vi "Create Wrapper for Code Module - Multiple Convertervi.vi"(11 "error in":errorcluster) -> (15 "error out":errorcluster)   [LabVIEW 2021, in "Converter.lvlib"]
uses:
  Converter.lvlib
  <vilib>/Utility/miscctls.llb/LVPointTypeDef.ctl
  <vilib>/Utility/traverseref.llb/TRef TravTarget.ctl
  <vilib>/Utility/traverseref.llb/VI Scripting - Traverse.lvlib
  Converter Reusables/Converter Reusables.lvlib
  Path Functions/Path Functions.lvlib
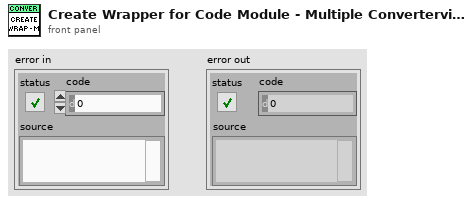
[diagram p1: front panel]
types:
  T1 = typedef "TRef TravTarget.ctl" = enum16{"FP", "BD", "Other"}
  T2 = typedef "LVPointTypeDef.ctl" = cluster{"Horizontal":i16, "Vertical":i16}
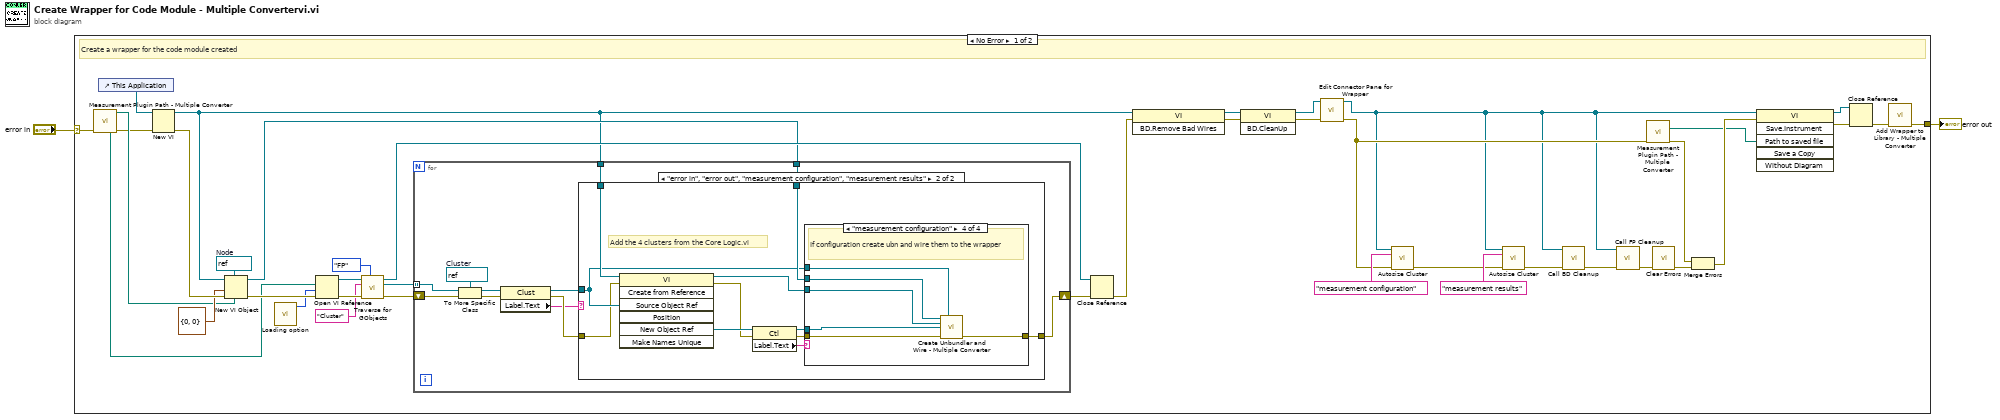
[diagram p0: block diagram]
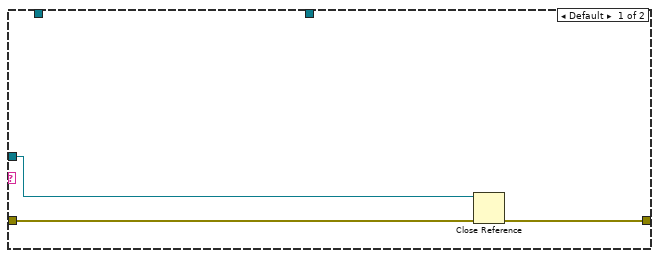
[diagram p2: hidden frame]
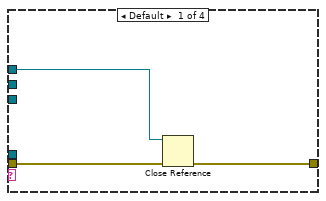
[diagram p3: hidden frame]
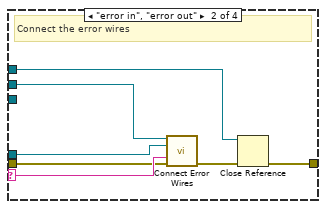
[diagram p4: hidden frame]
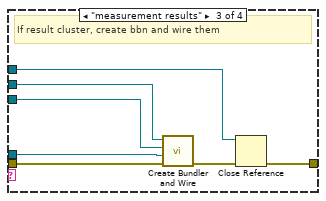
[diagram p5: hidden frame]
diagram:
  n1 = case shown="No Error" "error in" {
    selector: "error in" -> [w15 w92]
    tunnel: [w10 w92] -> w2
    frame No Error {
      w43 = refnum<vi> refnum  # Node
      # "Create a wrapper for the code module created"
      n2 = call "Measurement Plugin Path - Multiple Converter.vi"("error in"=w15) -> ("new code module"=w17:path, "logic vi path"=w16:path, "error out"=w14:errorcluster)  [unwired: 2 in, 10 out]
      n3 = control-ref of="This Application"() -> (w28:refnum<vi>)
      n4 = New VI(8:w14, 11:w28) -> (0:w42:errorcluster, 3:w27:refnum<vi>)  [unwired: 5 in]
      n5 = New VI Object(vi object class=w43, owner refnum=w27, position/next to=T2 {"Horizontal"=0, "Vertical"=0} ("location"), 6:w17, 8:w42) -> (object refnum=w29:refnum<vi>, 0:w38:errorcluster)  [unwired: 3 in]
      n6 = call "Loading option.vi"() -> ("options"=w3:i32)  [unwired: 11 in]
      n7 = Open VI Reference(vi path=w16, options=w3, error in (no error)=w38) -> (vi reference=w34:refnum<vi>, error out=w37:errorcluster)  [unwired: 3 in]
      n8 = call <vilib>:"Traverse for GObjects.vi"("Traverse Target"=TRef_TravTarget."FP", "error in (no error)"=w37, "Class Name"="Cluster", "VI Refnum"=w34) -> ("error out"=w35:errorcluster, "References"=w32:refnum<vi>[], "dup VI Refnum"=w31:refnum<vi>)  [unwired: 4 in, 1 out]
      n9 = for {
        shift-right: [w50] -> w33
        shift-left: w35 -> [w53]
        tunnel: w32 -> [w49] mode=indexing
        tunnel: w27 -> [w52]
        tunnel: w29 -> [w51]
        w54 = refnum<vi> refnum  # Cluster
        n10 = To More Specific Class(target class=w54, reference=w49, error in=w53) -> (specific class reference=w46:refnum<vi>, error out=w48:errorcluster)
        n11 = property class="Clust"(reference=w46, error in=w48) -> (reference out=w45:refnum<vi>, error out=w47:errorcluster, "Label.Text"=w44:string)
        n12 = case shown="\"error in\", \"error out\", \"measurement configuration\", \"measurement results\"" w44 {
          tunnel: w52 -> [_ w68]
          tunnel: w51 -> [_ w62]
          tunnel: [w56 w61] -> w50
          tunnel: w45 -> [w55 w59]
          tunnel: w47 -> [w57 w58]
          frame Default {
            n13 = Close Reference(reference=w55, error in (no error)=w57) -> (error out=w56:errorcluster)
          }
          frame "error in", "error out", "measurement configuration", "measurement results" {
            # "Add the 4 clusters from the Core Logic.vi"
            n14 = invoke class="VI" method="Create from Reference"(reference=w68, error in=w58, "Source Object Ref"=w59) -> (reference out=w63:refnum<vi>, error out=w66:errorcluster, "New Object Ref"=w67:refnum<vi>)  [unwired: 4 in, 4 out]
            n15 = property class="Ctl"(reference=w67, error in=w66) -> (reference out=w60:refnum<vi>, error out=w65:errorcluster, "Label.Text"=w64:string)
            n16 = case shown="\"measurement configuration\"" w64 {
              selector: w64 -> [_ w77 _ _]
              tunnel: w65 -> [w71 w74 w85 w87]
              tunnel: w63 -> [_ _ w84 w88]
              tunnel: w62 -> [_ w78 w83 w89]
              tunnel: [w69 w73 w81 w91] -> w61
              tunnel: w59 -> [w70 w72 w80 w90]
              tunnel: w60 -> [_ w75 w79 w86]
              frame Default {
                n17 = Close Reference(reference=w70, error in (no error)=w71) -> (error out=w69:errorcluster)
              }
              frame "error in", "error out" {
                # "Connect the error wires"
                n18 = call "Connect Error Wires.vi"("node in"=w78, "new object ref"=w75, "string"=w77, "error in"=w74) -> ("error out"=w76:errorcluster)  [unwired: 11 in]
                n19 = Close Reference(reference=w72, error in (no error)=w76) -> (error out=w73:errorcluster)
              }
              frame "measurement results" {
                # "If result cluster, create bbn and wire them"
                n20 = call "Create Bundler and Wire.vi"("error in"=w85, "new object ref"=w79, "vi refnum"=w84, "node ref"=w83) -> ("error out"=w82:errorcluster)  [unwired: 7 in]
                n21 = Close Reference(reference=w80, error in (no error)=w82) -> (error out=w81:errorcluster)
              }
              frame "measurement configuration" {
                # "If configuration create ubn and wire them to the wrapper"
                n22 = call "Create Unbundler and Wire - Multiple Converter.vi"("node in"=w89, "clust refnum"=w90, "vi refnum"=w88, "new object ref"=w86, "error in"=w87) -> ("error out"=w91:errorcluster)  [unwired: 10 in]
              }
            }
          }
        }
      }
      n23 = Close Reference(reference=w31, error in (no error)=w33) -> (error out=w24:errorcluster)
      n24 = invoke class="VI" method="BD.Remove Bad Wires"(reference=w27, error in=w24) -> (reference out=w26:refnum<vi>, error out=w25:errorcluster)  [unwired: 1 in, 1 out]
      n25 = invoke class="VI" method="BD.CleanUp"(reference=w26, error in=w25) -> (reference out=w19:refnum<vi>, error out=w18:errorcluster)  [unwired: 1 in, 1 out]
      n26 = call "Edit Connector Pane for Wrapper.vi"("vi reference in"=w19, "error in"=w18) -> ("vi reference out"=w4:refnum<vi>, "error out"=w7:errorcluster)  [unwired: 12 in]
      n27 = call "Autosize Cluster.vi"("vi refnum"=w4, "name"="measurement configuration" ("name/order"), "error in"=w7) -> ("error out"=w6:errorcluster)  [unwired: 12 in]
      n28 = call "Autosize Cluster.vi"("vi refnum"=w4, "name"="measurement results" ("name/order"), "error in"=w6) -> ("error out"=w5:errorcluster)  [unwired: 12 in]
      n29 = call "Call BD Cleanup.vi"("vi"=w4, "error in"=w5) -> ("error out"=w23:errorcluster)  [unwired: 13 in]
      n30 = call "Call FP Cleanup.vi"("vi"=w4, "error in"=w23) -> ("error out"=w22:errorcluster)  [unwired: 13 in]
      n31 = call "Measurement Plugin Path - Multiple Converter.vi"("error in"=w7) -> ("wrapper path"=w13:path, "error out"=w12:errorcluster)  [unwired: 2 in, 11 out]
      n32 = call <vilib>:"Clear Errors.vi"("error in (no error)"=w22) -> ("error out"=w21:errorcluster)  [unwired: 5 in, 1 out]
      n33 = Merge Errors(w12, w21) -> (w20:errorcluster)
      n34 = invoke class="VI" method="Save.Instrument"(reference=w4, error in=w20, "Path to saved file"=w13) -> (reference out=w39:refnum<vi>, error out=w40:errorcluster)  [unwired: 3 in, 4 out]
      n35 = Close Reference(reference=w39, error in (no error)=w40) -> (error out=w11:errorcluster)
      n36 = call "Add Wrapper to Library - Multiple Converter.vi"("error in"=w11) -> ("error out"=w10:errorcluster)  [unwired: 14 in]
    }
    frame Error {
    }
  }
  "error out" <- w2
